vi "RemoteVI Check Tips Message.vi"() -> (4 "labels":string[](array[string]), 6 "expected":string[](array[string]), 8 "actual":string[](array[string]), 10 "failures":i32)   [LabVIEW 2020]
doc: "Test support, generated by tests/caraya/build.py from tests/vectors/text.json (tips) - do not edit. Calls RemoteVI Tips Message.vi once per vector: each tip's text is the vector's code units as bytes (all below 0x100); the message is compared as the string it is. Outputs, one element per vector: labels (the vector's name), expected (rendered from the vector), actual (the VI's result rendered the same way), and failures, the number of vectors whose expected and actual differ."
uses:
  source/RemoteVI.lvlib
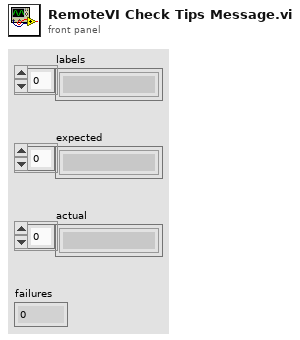
[diagram p1: front panel]
types:
  T1 = cluster{"name":string, "tips":cluster{"x":i32, "y":i32, "w":i32, "h":i32, "text":string}[], "expect":string}[]
  T2 = cluster{"x":i32, "y":i32, "w":i32, "h":i32, "text":string}[]
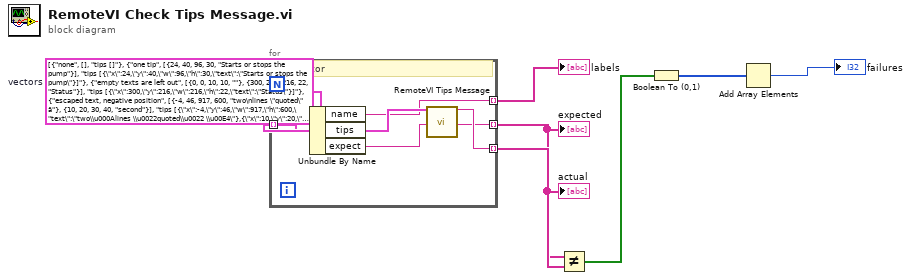
[diagram p0: block diagram]
diagram:
  w1 = T1 [{"name"="none", "tips"=[], "expect"="tips []"}, {"name"="one tip", "tips"=[{"x"=24, "y"=40, "w"=96, "h"=30, "text"="Starts or stops the pump"}], "expect"="tips [{\"x\":24,\"y\":40,\"w\":96,\"h\":30,\"text\":\"Starts or stops the pump\"}]"}, {"name"="empty texts are left out", "tips"=[{"x"=0, "y"=0, "w"=10, "h"=10, "text"=""}, {"x"=300, "y"=216, "w"=216, "h"=22, "text"="Status"}], "expect"="tips [{\"x\":300,\"y\":216,\"w\":216,\"h\":22,\"text\":\"Status\"}]"}, {"name"="escaped text, negative position", "tips"=[{"x"=-4, "y"=46, "w"=917, "h"=600, "text"="two\nlines \"quoted\" ä"}, {"x"=10, "y"=20, "w"=30, "h"=40, "text"="second"}], "expect"="tips [{\"x\":-4,\"y\":46,\"w\":917,\"h\":600,\"text\":\"two\\u000Alines \\u0022quoted\\u0022 \\u00E4\"},{\"x\":10,\"y\":20,\"w\":30,\"h\":40,\"text\":\"second\"}]"}]  # vectors
  n1 = for {
    tunnel: w1 -> [w8] mode=indexing
    tunnel: [w9] -> w2 mode=indexing
    tunnel: [w11] -> w3 mode=indexing
    tunnel: [w12] -> w4 mode=indexing
    # "One vector"
    n2 = Unbundle By Name(w8) -> ("name"=w9:string, "tips"=w10:T2, "expect"=w11:string)
    n3 = call "RemoteVI Tips Message.vi"("tips"=w10) -> ("message"=w12:string)  [unwired: 14 in]
  }
  "labels" <- w2
  "expected" <- w3
  "actual" <- w4
  n4 = Not Equal?(x=w3, y=w4) -> (x != y?=w5:bool[])
  n5 = Boolean To (0,1)(Boolean=w5) -> (0, 1=w6:i16[])
  n6 = Add Array Elements(numeric array=w6) -> (sum=→"failures":i16)
